vi "CreateCommandWrapper.vi"() -> ()   [LabVIEW 2025]
doc: "Creates a reentrant command wrapper. Wires all subVI inputs/outputs to named controls/indicators. No connector assignments. Never executes the command."
uses:
  <vilib>/Utility/miscctls.llb/LVPointTypeDef.ctl
panel:
  out "error out":errorcluster
  out "terminal errors":errorcluster[](array[cluster])
  in  "terminal numbers":dbl[](array[numeric])
  in  "wrapper path":string
  in  "command path":string
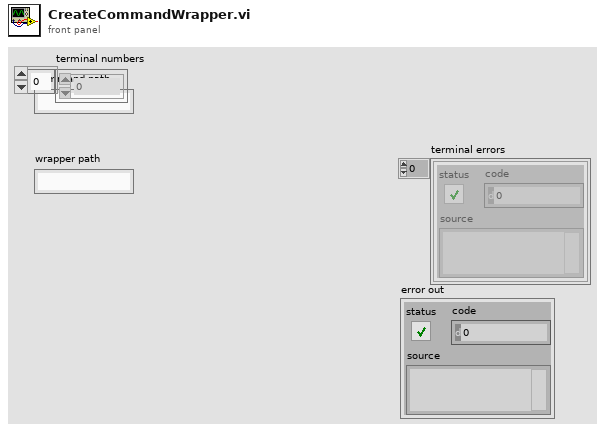
[diagram p1: front panel]
types:
  T1 = typedef "LVPointTypeDef.ctl" = cluster{"Horizontal":i16, "Vertical":i16}
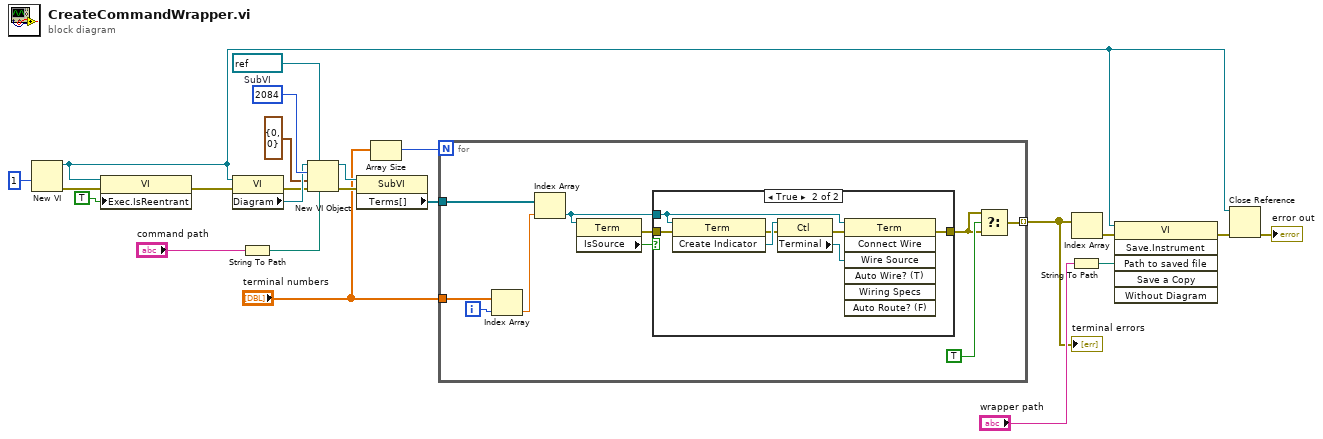
[diagram p0: block diagram]
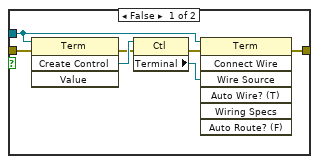
[diagram p2: hidden frame]
diagram:
  w16 = refnum<vi> refnum  # SubVI
  n1 = New VI(9:1) -> (0:w19:errorcluster, 3:w20:refnum<vi>)  [unwired: 6 in]
  n2 = property class="VI"(reference=w20, error in=w19, "Exec.IsReentrant"=TRUE) -> (error out=w17:errorcluster)  [unwired: 1 out]
  n3 = property class="VI"(reference=w20, error in=w17) -> (error out=w13:errorcluster, "Diagram"=w14:refnum<vi>)  [unwired: 1 out]
  n4 = String To Path(string="command path") -> (path=w12:path)
  n5 = New VI Object(vi object class=w16, owner refnum=w14, style=u32 2084, position/next to=T1 {"Horizontal"=0, "Vertical"=0} ("location"), 6:w12, 8:w13) -> (object refnum=w10:refnum<vi>, 0:w9:errorcluster)  [unwired: 2 in]
  n6 = property class="SubVI"(reference=w10, error in=w9) -> ("Terms[]"=w6:refnum<vi>[])  [unwired: 2 out]
  n7 = Array Size(array="terminal numbers") -> (size(s)=w8:i32)
  n8 = for {
    N: w8 -> [_]
    tunnel: "terminal numbers" -> [w33]
    tunnel: w6 -> [w31]
    tunnel: [w24] -> w5 mode=indexing
    i -> [w32]
    n9 = Index Array(array=w33, index=w32) -> (element=w30:dbl)
    n10 = Index Array(array=w31, index=w30) -> (element=w28:refnum<vi>)
    n11 = property class="Term"(reference=w28) -> (error out=w27:errorcluster, "IsSource"=w29:bool)  [unwired: 1 in, 1 out]
    n12 = case shown="True" w29 {
      tunnel: w28 -> [w40 w47]
      tunnel: w27 -> [w39 w46]
      tunnel: [w34 w41] -> w25
      frame False {
        n13 = invoke class="Term" method="Create Control"(reference=w40, error in=w39) -> (error out=w37:errorcluster, "Create Control"=w38:refnum<vi>)  [unwired: 2 in, 2 out]
        n14 = property class="Ctl"(reference=w38, error in=w37) -> (error out=w36:errorcluster, "Terminal"=w35:refnum<vi>)  [unwired: 1 out]
        n15 = invoke class="Term" method="Connect Wire"(reference=w40, error in=w36, "Wire Source"=w35) -> (error out=w34:errorcluster)  [unwired: 4 in, 6 out]
      }
      frame True {
        n16 = invoke class="Term" method="Create Indicator"(reference=w47, error in=w46) -> (error out=w44:errorcluster, "Create Indicator"=w45:refnum<vi>)  [unwired: 1 in, 1 out]
        n17 = property class="Ctl"(reference=w45, error in=w44) -> (error out=w43:errorcluster, "Terminal"=w42:refnum<vi>)  [unwired: 1 out]
        n18 = invoke class="Term" method="Connect Wire"(reference=w47, error in=w43, "Wire Source"=w42) -> (error out=w41:errorcluster)  [unwired: 4 in, 6 out]
      }
    }
    n19 = Select(t=w25, s=TRUE, f=w25) -> (s? t:f=w24:errorcluster)
  }
  "terminal errors" <- w5
  n20 = String To Path(string="wrapper path") -> (path=w3:path)
  n21 = Index Array(array=w5) -> (element=w4:errorcluster)  [unwired: 1 in]
  n22 = invoke class="VI" method="Save.Instrument"(reference=w20, error in=w4, "Path to saved file"=w3) -> (error out=w2:errorcluster)  [unwired: 3 in, 5 out]
  n23 = Close Reference(reference=w20, error in (no error)=w2) -> (error out=→"error out":errorcluster)
